vi "SetDevice.vi"(8 "error in":errorcluster, 11 "Index":i32) -> (0 "error out":errorcluster)   [LabVIEW 2020, in "OpenLvVision_OpenCv.lvlib" / "Cuda.lvlib"]
doc: "Sets a device and initializes it for the current thread."
uses:
  Cuda.lvlib
  OpenLvVision_OpenCv.lvlib
  Dlls/OlvOpenCvWrapper.dll
  <vilib>/Utility/error.llb/Error Cluster From Error Code.vi
  <vilib>/ErrorRing/Error Ring.xnode
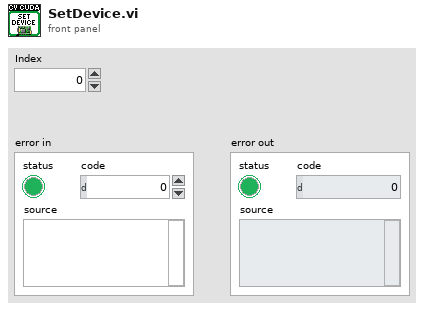
[diagram p1: front panel]
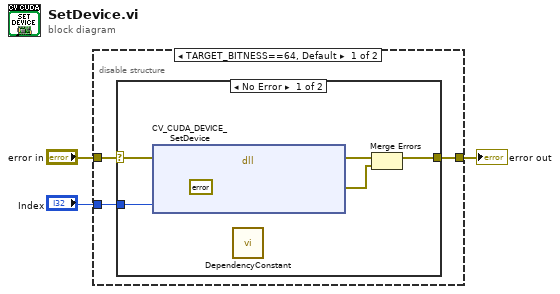
[diagram p0: block diagram]
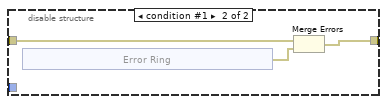
[diagram p3: hidden frame]
diagram:
  n1 = disable-structure shown="TARGET_BITNESS==64, Default" {
    disable-tunnel: "error in" -> [w5 w16]
    disable-tunnel: [w6 w15] -> w2
    disable-tunnel: "Index" -> [w4 _]
    frame condition #0 (active) {
      n2 = case shown="No Error" w5 {
        selector: w5 -> [w8 w13]
        tunnel: [w9 w13] -> w6
        tunnel: w4 -> [w7 _]
        frame No Error {
          n3 = dll-call lib="C:/Users/lukas/Documents/OpenLvVision_OpenCv/SourceCode/LabView/OpenLvVision_OpenCv/Dlls/OlvOpenCvWrapper.dll" fn="CV_CUDA_DEVICE_SetDevice"(error in=w8, "Error"=errorcluster {"status"=FALSE, "code"=0, "source"=""} ("error out"), "index"=w7) -> (error out=w12:errorcluster, "Error"=w11:errorcluster)  [unwired: 4 in, 1 out]
          n4 = call "DependencyConstant.vi"() -> ()  [unwired: 12 in]
          n5 = Merge Errors(w12, w11) -> (w9:errorcluster)
        }
        frame Error {
        }
      }
    }
    frame condition #1 {
      n6 = xnode "Error Ring"() -> ("error out"=w14:errorcluster)
      n7 = Merge Errors(w16, w14) -> (w15:errorcluster)
    }
  }
  "error out" <- w2
